vi "Assert False.vi"(4 "Execution time (s)":dbl=-1.0, 5 "Assert Only? (F)":bool, 6 "error code (1)":i32=1, 7 "Label":string, 8 "error in (no error)":errorcluster, 9 "Register with caller test (F)":bool, 11 "False?":bool) -> (0 "error out":errorcluster, 2 "Properties.Assert":refnum<class "Properties.Assert.lvclass">)   [LabVIEW 2020, in "Caraya.lvlib" / "Assert.lvclass"]
doc: "Generates an error if the input condition is not met.\n\n--\nCopyright © 2015 JKI All rights reserved.\n\nAuthor: Tomi Maila <tomi.maila@jki.net>\n\nThis library is provided \"AS IS\" ,WITHOUT WARRANTIES OR\nCONDITIONS OF ANY KIND, either express or implied.\n\nJKI -- jki.net"
uses:
  Assert.lvclass
  Properties.Assert/Properties.Assert.lvclass
  C:/projects/caraya/src/classes/Properties/Properties.lvclass
  Properties/Properties.lvclass
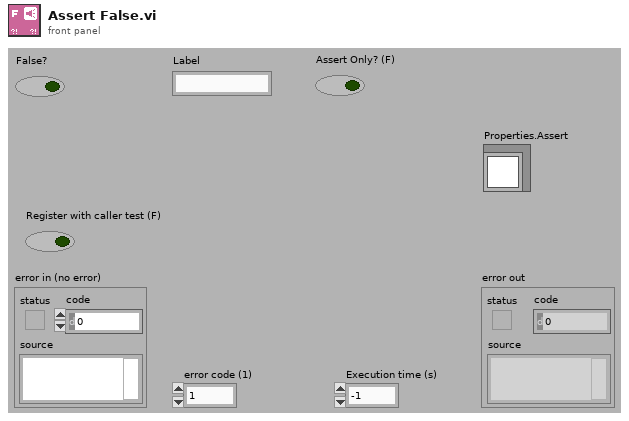
[diagram p1: front panel]
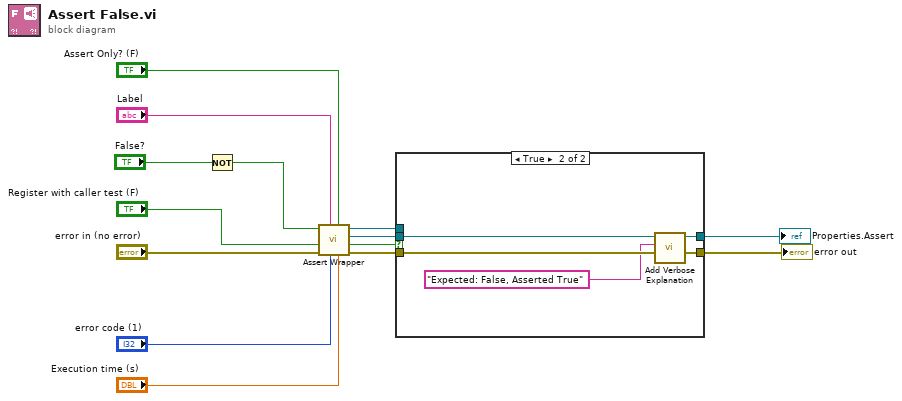
[diagram p0: block diagram]
diagram:
  n1 = Not(x="False?") -> (.not. x?=w11:bool)
  n2 = call "Assert Wrapper.vi"("Execution time (s)"="Execution time (s)", "Assert Only? (F)"="Assert Only? (F)", "error code (1)"="error code (1)", "Label"="Label", "error in (no error)"="error in (no error)", "Register with caller test (F)"="Register with caller test (F)", "Assert?"=w11) -> ("error out"=w6:errorcluster, "Verbose"=w5:bool, "Properties.Assert"=w2:refnum<class "Properties.Assert.lvclass">, "Assert out"=w3:refnum<class "Assert.lvclass">)  [unwired: 1 in]
  n3 = case shown="True" w5 {
    tunnel: [w16 w20] -> w8
    tunnel: w3 -> [_ _]
    tunnel: w6 -> [w16 w21]
    tunnel: w2 -> [w15 w18]
    tunnel: [w15 w17] -> w1
    frame False {
    }
    frame True {
      n4 = call "Add Verbose Explanation.vi"("error in (no error)"=w21, "Verbose Explanation"="Expected: False, Asserted True", "Properties"=w18) -> ("error out"=w20:errorcluster, "Properties"=w17:refnum<class "Properties.Assert.lvclass">)  [unwired: 7 in]
    }
  }
  "error out" <- w8
  "Properties.Assert" <- w1
